vi "DUT Bring Up.vi"(8 "error in":errorcluster, 9 "DPI Instrument Name":refnum<k15>, 10 "DUT Bring Up":string, 11 "DPE Project File Path":string) -> (0 "error out":errorcluster, 1 "DUT Bring Up Vcc Resource":refnum<k15>[](array[refnum]), 2 "DUT Bring Up DCPower Channels":string[](array[string]), 3 "DUT Bring Up PASS?":bool, 5 "DPI Instrument Name":refnum<k15>, 7 "DUT Bring Up Pin":string[](array[string]))   [LabVIEW 2025, in "Digital Pattern Sequencer.lvclass"]
uses:
  Digital Pattern Sequencer.lvclass
  Digital Pattern Sequencer.lvclass/Digital Pattern Sequencer.ctl
  <instrlib>/niDCPower/nidcpower.llb/niDCPower Source Mode.ctl
  <instrlib>/niDCPower/nidcpower.llb/niDCPower Output Function.ctl
  <instrlib>/niDCPower/nidcpower.llb/niDCPower Wait For Event - Event.ctl
  <instrlib>/niDigital/niDigital.llb/niDigital Measurement Type.ctl
  <instrlib>/niDCPower/nidcpower.llb/niDCPower Get Channel Name From String.vi
  <instrlib>/niDigital/niDigital.llb/niDigital Burst Pattern (Pass Fail).vi
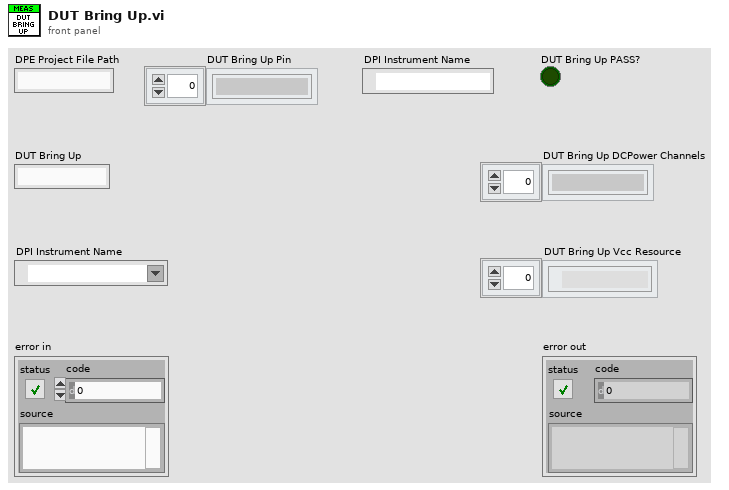
[diagram p1: front panel]
types:
  T1 = typedef "niDigital Measurement Type.ctl" = i32
  T2 = typedef "niDCPower Wait For Event - Event.ctl" = i32
  T3 = typedef "niDCPower Output Function.ctl" = i32
  T4 = typedef "niDCPower Source Mode.ctl" = i32
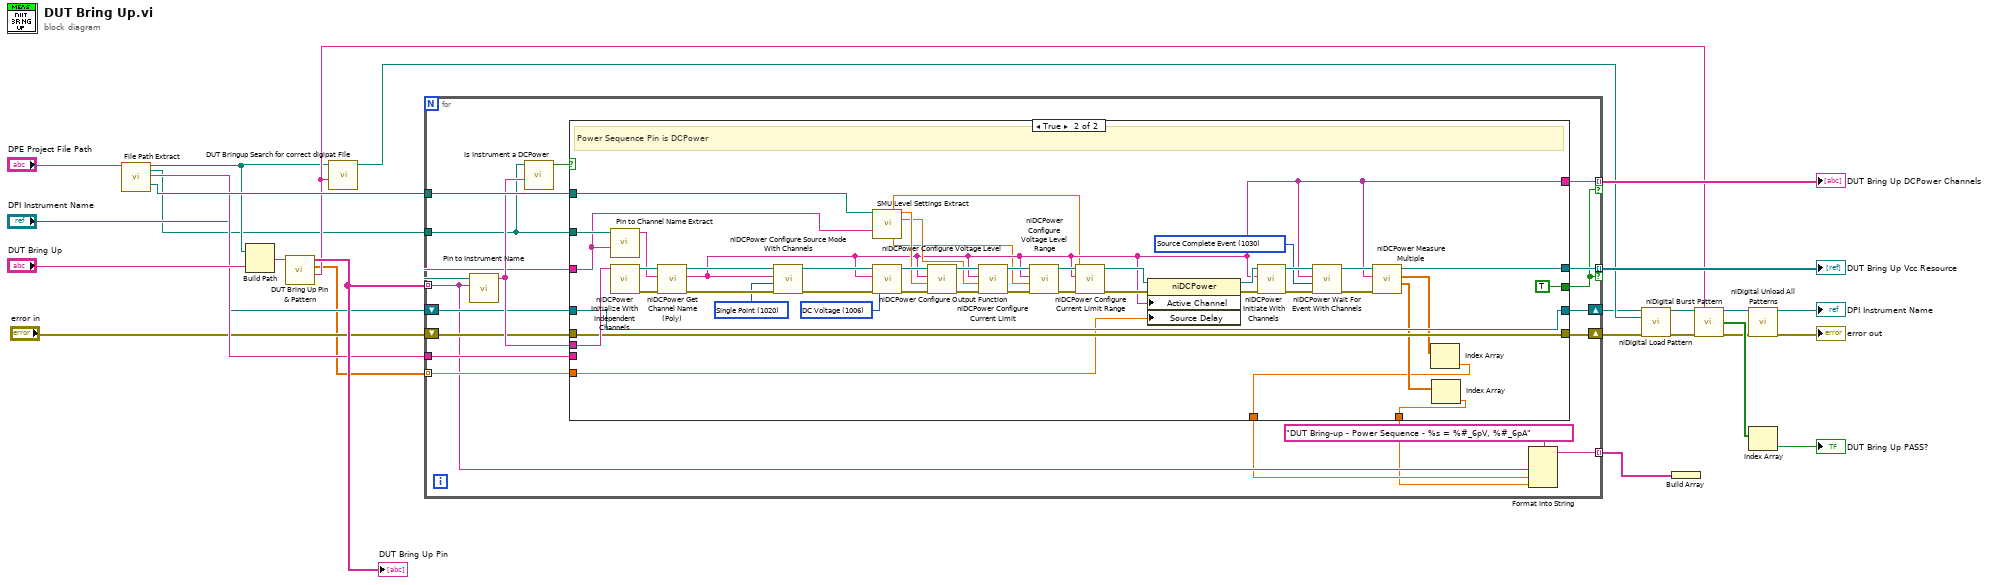
[diagram p0: block diagram]
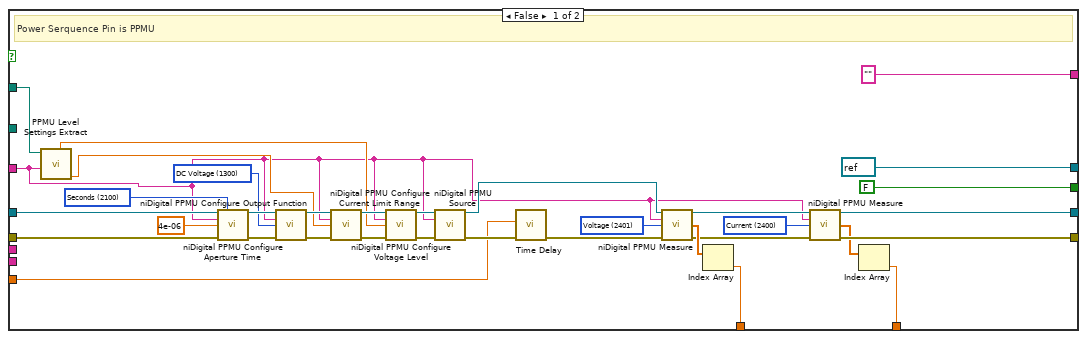
[diagram p2: hidden frame]
diagram:
  n1 = call "File Path Extract.vi"("DPE Project File Path"="DPE Project File Path") -> ("DPE Project Path"=w14:path, ".pinmap file path"=w3:path, "DPI Instrument Name"=w12:string, ".digilevels file path"=w20:path)  [unwired: 10 in, 5 out]
  n2 = Build Path(base path=w14, name or relative path="DUT Bring Up") -> (appended path=w21:path)
  n3 = call "DUT Bring Up Pin & Pattern.vi"(".dutbringup File Path"=w21) -> ("Bring-up Pattern"=w15:string, "Post Source Delay"=w2:dbl[], "Power Sequence Pins"=w24:string[])  [unwired: 8 in]
  "DUT Bring Up Pin" <- w24
  n4 = call "DUT Bringup Search for correct digipat File.vi"("DUT Bring Up Pattern name"=w15, "DPE Project Path"=w14) -> ("DUT Bring Up .digipat File"=w13:path)  [unwired: 8 in]
  n5 = for {
    tunnel: w24 -> [w30] mode=indexing
    tunnel: w20 -> [w44]
    tunnel: [w43] -> w17 mode=indexing if=w33
    tunnel: [w42] -> w16 mode=indexing if=w33
    tunnel: w12 -> [w39]
    tunnel: w3 -> [w34]
    shift-right: [w36] -> w5
    shift-left: "DPI Instrument Name" -> [w38]
    shift-right: [w35] -> w4
    shift-left: "error in" -> [w37]
    tunnel: w2 -> [w32] mode=indexing
    tunnel: [w27] -> w1 mode=indexing
    n6 = call "Pin to Instrument Name.vi"(".pinmap File Path"=w34, "Pin Name"=w30) -> ("Instrument Name"=w40:string)  [unwired: 8 in]
    n7 = call "Is Instrument a DCPower.vi"("Instrument Name"=w40, ".pinmap File Path"=w34) -> ("DCPower?"=w41:bool)  [unwired: 9 in]
    n8 = case shown="True" w41 {
      tunnel: w40 -> [_ w99]
      tunnel: w30 -> [w49 w84]
      tunnel: w34 -> [_ w87]
      tunnel: w44 -> [w68 w93]
      tunnel: [w50 w86] -> w36
      tunnel: [w52 w85] -> w35
      tunnel: [refnum<k15> refnum ("instrument handle out") w92] -> w42
      tunnel: ["" ("name") w91] -> w43
      tunnel: [FALSE TRUE] -> w33
      tunnel: w39 -> [_ _]
      tunnel: w38 -> [w55 w86]
      tunnel: w37 -> [w54 w85]
      tunnel: w32 -> [w53 w83]
      tunnel: [w46 w80] -> w29
      tunnel: [w45 w79] -> w28
      frame False {
        w48 = T1 2400 items=["Voltage"=2401, "Current"=2400] ("measurement type")
        w76 = u16 2401 items=["Voltage"=2401, "Current"=2400] ("measurement type")
        w77 = u16 2100 items=["Seconds"=2100] ("aperture time units")
        w71 = u16 1300 items=["DC Voltage"=1300, "DC Current"=1301] ("output function")
        # "Power Serquence Pin is PPMU"
        n9 = call "PPMU Level Settings Extract.vi"("Pin Name"=w49, ".digilevel File Path"=w68) -> ("IRange"=w57:dbl, "Vf"=w56:dbl)  [unwired: 5 in, 3 out]
        n10 = call <instrlib>:"niDigital PPMU Configure Aperture Time.vi"("instrument handle"=w55, "aperture time units"=w77, "channel list"=w49, "aperture time"=4e-06, "error in"=w54) -> ("instrument handle out"=w75:refnum<k15>, "error out"=w74:errorcluster)  [unwired: 9 in]
        n11 = call <instrlib>:"niDigital PPMU Configure Output Function.vi"("instrument handle"=w75, "channel list"=w49, "output function"=w71, "error in"=w74) -> ("instrument handle out"=w63:refnum<k15>, "error out"=w60:errorcluster)  [unwired: 10 in]
        n12 = call <instrlib>:"niDigital PPMU Configure Current Limit Range.vi"("instrument handle"=w63, "channel list"=w49, "current limit range (A)"=w57, "error in"=w60) -> ("instrument handle out"=w62:refnum<k15>, "error out"=w59:errorcluster)  [unwired: 10 in]
        n13 = call <instrlib>:"niDigital PPMU Configure Voltage Level.vi"("instrument handle"=w62, "channel list"=w49, "voltage level (V)"=w56, "error in"=w59) -> ("instrument handle out"=w61:refnum<k15>, "error out"=w58:errorcluster)  [unwired: 10 in]
        n14 = call <instrlib>:"niDigital PPMU Source.vi"("instrument handle"=w61, "channel list"=w49, "error in"=w58) -> ("instrument handle out"=w78:refnum<k15>, "error out"=w70:errorcluster)  [unwired: 11 in]
        n15 = call "Time Delay"("error in (no error)"=w70, "Delay Time (s)"=w53) -> ("error out"=w72:errorcluster)  [unwired: 9 in]
        n16 = call <instrlib>:"niDigital PPMU Measure.vi"("instrument handle"=w78, "channel list"=w49, "measurement type"=w76, "error in"=w72) -> ("instrument handle out"=w51:refnum<k15>, "measurements"=w69:dbl[], "error out"=w67:errorcluster)  [unwired: 9 in]
        n17 = Index Array(array=w69) -> (element=w46:dbl)  [unwired: 1 in]
        n18 = call <instrlib>:"niDigital PPMU Measure.vi"("instrument handle"=w51, "channel list"=w49, "measurement type"=w48, "error in"=w67) -> ("instrument handle out"=w50:refnum<k15>, "measurements"=w47:dbl[], "error out"=w52:errorcluster)  [unwired: 9 in]
        n19 = Index Array(array=w47) -> (element=w45:dbl)  [unwired: 1 in]
      }
      frame True {
        w97 = T2 1030 items=["Source Complete Event"=1030, "Measure Complete Event"=1031, "Sequence Iteration Complete Event"=1032, "Sequence Engine Done Event"=1033] ("event")
        w100 = T3 1006 items=["DC Voltage"=1006, "DC Current"=1007, "Pulse Voltage"=1049, "Pulse Current"=1050] ("output function")
        w98 = T4 1020 items=["Single Point"=1020, "Sequence"=1021] ("source mode")
        # "Power Sequence Pin is DCPower"
        n20 = call "Pin to Channel Name Extract.vi"(".pinmap File Path"=w87, "Pin Name"=w84) -> ("Channel"=w94:string)  [unwired: 8 in]
        n21 = call <instrlib>:"niDCPower Initialize With Independent Channels.vi"("resource name"=w99) -> ("error out"=w121:errorcluster, "instrument handle out"=w103:refnum<k15>)  [unwired: 9 in]
        n22 = call-poly <instrlib>:"niDCPower Get Channel Name (Poly).vi"("error in (no error)"=w121, "index"=w94, "instrument handle"=w103) -> ("error out"=w122:errorcluster, "name"=w91:string, "instrument handle out"=w120:refnum<k15>)  [unwired: 6 in]
        n23 = call <instrlib>:"niDCPower Configure Source Mode With Channels.vi"("error in (no error)"=w122, "source mode"=w98, "channel name"=w91, "instrument handle"=w120) -> ("error out"=w104:errorcluster, "instrument handle out"=w105:refnum<k15>)  [unwired: 6 in]
        n24 = call "SMU Level Settings Extract.vi"(".digilevel File Path"=w93, "Pin Name"=w84) -> ("IRange"=w89:dbl, "Vf"=w96:dbl, "Ic"=w95:dbl, "VRange"=w88:dbl)  [unwired: 7 in, 3 out]
        n25 = call <instrlib>:"niDCPower Configure Output Function.vi"("error in (no error)"=w104, "output function"=w100, "channel name"=w91, "instrument handle"=w105) -> ("error out"=w119:errorcluster, "instrument handle out"=w118:refnum<k15>)  [unwired: 6 out]
        n26 = call <instrlib>:"niDCPower Configure Voltage Level.vi"("error in (no error)"=w119, "voltage level"=w96, "channel name"=w91, "instrument handle"=w118) -> ("error out"=w102:errorcluster, "instrument handle out"=w101:refnum<k15>)  [unwired: 6 out]
        n27 = call <instrlib>:"niDCPower Configure Current Limit.vi"("error in (no error)"=w102, "current limit"=w95, "channel name"=w91, "instrument handle"=w101) -> ("error out"=w106:errorcluster, "instrument handle out"=w107:refnum<k15>)  [unwired: 1 in, 5 out]
        n28 = call <instrlib>:"niDCPower Configure Voltage Level Range.vi"("error in (no error)"=w106, "voltage level range"=w88, "channel name"=w91, "instrument handle"=w107) -> ("error out"=w108:errorcluster, "instrument handle out"=w109:refnum<k15>)  [unwired: 6 out]
        n29 = call <instrlib>:"niDCPower Configure Current Limit Range.vi"("error in (no error)"=w108, "current limit range"=w89, "channel name"=w91, "instrument handle"=w109) -> ("error out"=w113:errorcluster, "instrument handle out"=w110:refnum<k15>)  [unwired: 6 out]
        n30 = property class="niDCPower"(reference=w110, error in=w113, "Active Channel"=w91, "Source Delay"=w83) -> (reference out=w111:refnum<k15>, error out=w112:errorcluster)
        n31 = call <instrlib>:"niDCPower Initiate With Channels.vi"("error in (no error)"=w112, "channel name"=w91, "instrument handle"=w111) -> ("error out"=w116:errorcluster, "instrument handle out"=w114:refnum<k15>)  [unwired: 7 in]
        n32 = call <instrlib>:"niDCPower Wait For Event With Channels.vi"("error in (no error)"=w116, "event"=w97, "channel name"=w91, "instrument handle"=w114) -> ("error out"=w117:errorcluster, "instrument handle out"=w115:refnum<k15>)  [unwired: 6 in]
        n33 = call <instrlib>:"niDCPower Measure Multiple.vi"("error in (no error)"=w117, "channel name"=w91, "instrument handle"=w115) -> ("current measurements"=w81:dbl[], "voltage measurements"=w82:dbl[], "instrument handle out"=w92:refnum<k15>)  [unwired: 6 out]
        n34 = Index Array(array=w82) -> (element=w80:dbl)  [unwired: 1 in]
        n35 = Index Array(array=w81) -> (element=w79:dbl)  [unwired: 1 in]
      }
    }
    n36 = Format Into String(format string="DUT Bring-up - Power Sequence - %s = %#_6pV, %#_6pA", w30, w29, w28) -> (resulting string=w27:string)  [unwired: 2 in, 1 out]
  }
  "DUT Bring Up DCPower Channels" <- w17
  "DUT Bring Up Vcc Resource" <- w16
  n37 = call <instrlib>:"niDigital Load Pattern.vi"("instrument handle"=w5, "pattern file"=w13, "error in"=w4) -> ("instrument handle out"=w26:refnum<k15>, "error out"=w25:errorcluster)  [unwired: 11 in]
  n38 = Build Array(w1) -> ()  [unwired: 1 out]
  n39 = call-poly <instrlib>:"niDigital Burst Pattern.vi"("instrument handle"=w26, "start label"=w15, "error in"=w25) -> ("instrument handle out"=w10:refnum<k15>, "pass"=w19:bool[], "error out"=w9:errorcluster)  [unwired: 10 in]
  n40 = call <instrlib>:"niDigital Unload All Patterns.vi"("instrument handle"=w10, "error in"=w9) -> ("instrument handle out"=→"DPI Instrument Name":refnum<k15>, "error out"=→"error out":errorcluster)  [unwired: 12 in]
  n41 = Index Array(array=w19) -> (element=→"DUT Bring Up PASS?":bool)  [unwired: 1 in]
